vi "MUX - Switch Control.vi"() -> ()   [LabVIEW 2013]
doc: "Sample numeric display item."
uses:
  <vilib>/NI Veristand/Display Template Support/Display Template Support.llb/cluster_Screen Item Settings.ctl
  <vilib>/NI Veristand/Display Template Support/Display Template Support.llb/cluster_Graph Scale Settings.ctl
  <vilib>/NI Veristand/Display Template Support/Display Template Support.llb/cluster_Graph Plot Settings.ctl
  NationalInstruments.VeriStand.SystemStorage
  SubVIs/Relay Data.ctl
  SubVIs/Switch.ctl
  <vilib>/NI Veristand/Display Template Support/Display Template Support.llb/enum_Display Template Handler Minimal To Widget Msg.ctl
  <vilib>/NI Veristand/Display Template Support/Display Template Support.llb/enum_Display Template Handler Minimal To Workspace.ctl
  <vilib>/NI Veristand/Display Template Support/Display Template Support.llb/sub_Display Template Handler Custom.vi
  <vilib>/NI Veristand/Execution/Workspace/NI_VS Workspace ExecutionAPI.lvlib
  MUX Custom Device.lvlib
panel:
  out "MUX Name":string
  in  "Open":bool
  in  "Relays":T1[](array[typedef])
  in  "NIVS.Gateway IP Address":string
  in  "NIVS.System Definition Root":refnum<k24>
  in  "Item.Data":T3
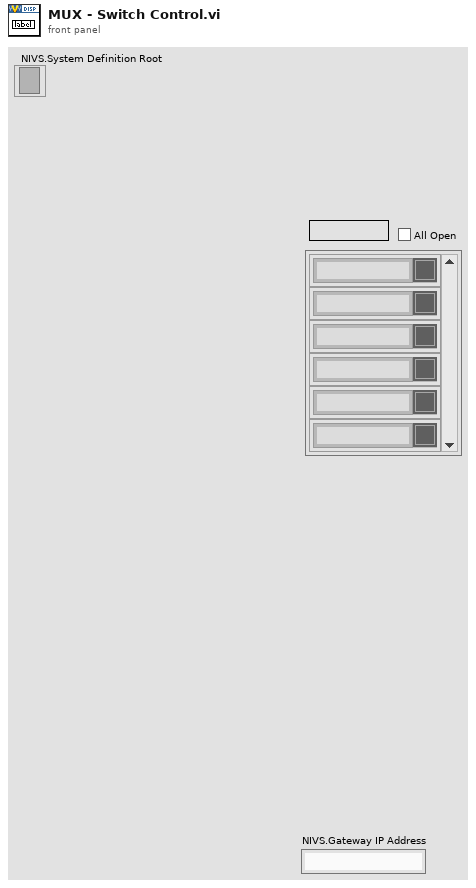
[diagram p1: front panel]
types:
  T1 = typedef "MUX Custom Device.lvlib/Relay Data.ctl" = cluster{"Relay Name":string, "State":T2}
  T2 = typedef "MUX Custom Device.lvlib/Switch.ctl" = bool
  T3 = typedef "cluster_Screen Item Settings.ctl" = cluster{"Template VI":string, "Position X":i32, "Position Y":i32, "Custom":string, "Show Title Bar":bool, "ID":i32, "Always On Top":bool, "Allow Resize":bool, "Allow Minimize":bool, "Allow Close":bool, "Size to Screen":bool, "Screen.ID":i32, "State":enum16{"Normal", "New"}, "Title":string, "Window Bounds":cluster{"[0]":i16, "[1]":i16, "[2]":i16, "[3]":i16}, "Channel Ref":u64, "Unit":string, "Default Units?":bool, "Flash Limit?":bool, "Color 1":u32, "Color 2":u32, "Color 3":u32, "Color 4":u32, "Bck Color":u32, "Fore Color":u32, "Limit 1":dbl, "Limit 2":dbl, "Limit 3":dbl, "Limit 4":dbl, "Limit Mode 1":i32, "Limit Mode 2":i32, "Limit Mode 3":i32, "Limit Mode 4":i32, "Scale Precision":i32, "Scale Min":dbl, "Scale Max":dbl, "Format":i32, "Precision":i32, "Background Type":i32, "IDs":i32[], "Units":string[], "Labels":string[], "Scale Factor":dbl, "Scale Offset":dbl, "YScale Index":u32[], "XScale":T4, "YScales":T4[], "Plots":T5[], "Update Period":dbl, "History Length":dbl, "My.Ref":refnum<vi>, "Is Control?":bool, "Channel Paths":string[], "Custom Data":variant}
  T4 = typedef "cluster_Graph Scale Settings.ctl" = cluster{"Format":u8, "Precision":u8, "Fit":u8, "Label":string, "Use Default Label":bool, "Label Visible":bool, "Min":dbl, "Max":dbl}
  T5 = typedef "cluster_Graph Plot Settings.ctl" = cluster{"Bar Style":u8, "Fill To":i16, "Fill/PtColor":u32, "Line Style":u8, "Line Width":u8, "Color":u32, "Interp":u8, "Point Style":u8}
  T6 = typedef "enum_Display Template Handler Minimal To Workspace.ctl" = cluster{"Operation":enum16{"SetCustomData", "DeleteItem"}, "Data":variant}
  T7 = typedef "enum_Display Template Handler Minimal To Widget Msg.ctl" = enum16{"Stop", "LaunchConfigDialog"}
  T8 = typedef "NI_VS Workspace ExecutionAPI.lvlib/WorkspaceAPI.ctl" = refnum<k24>
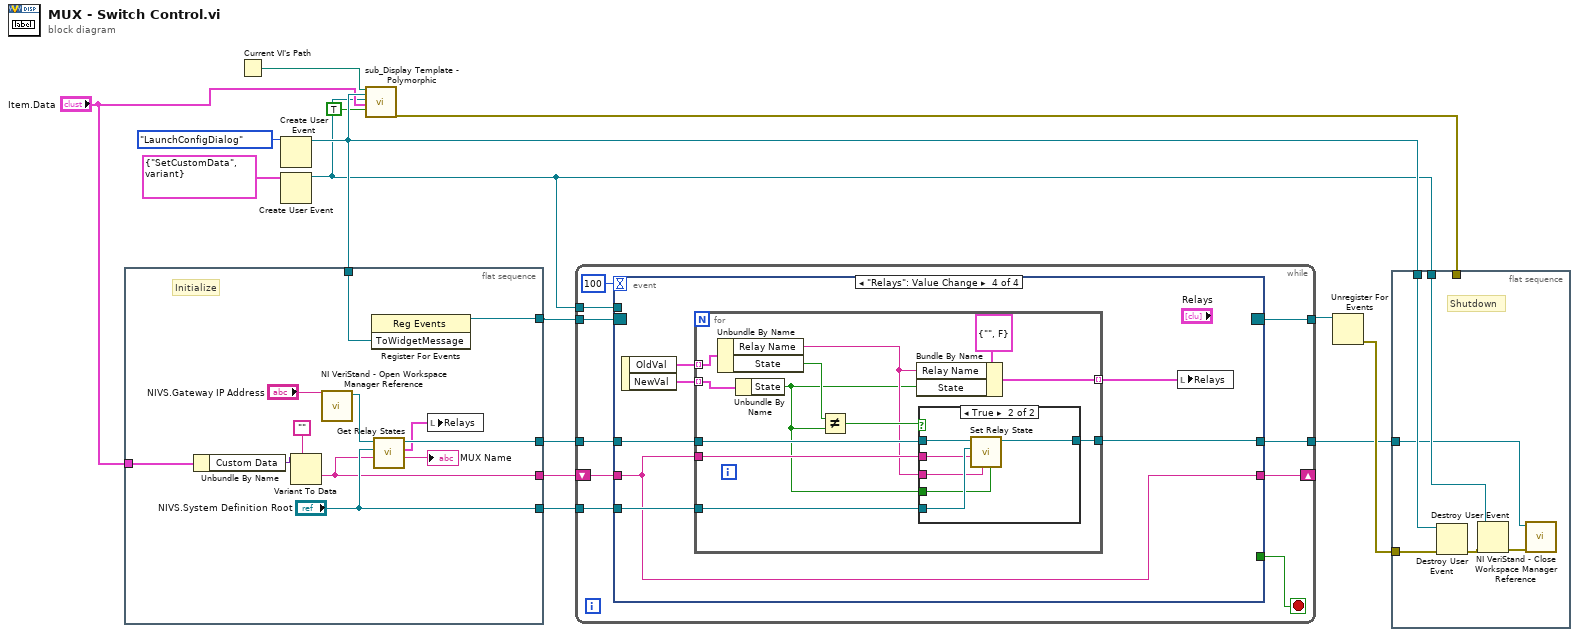
[diagram p0: block diagram]
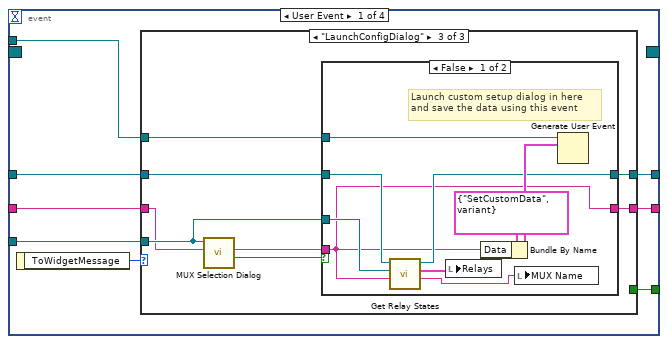
[diagram p2: hidden frame]
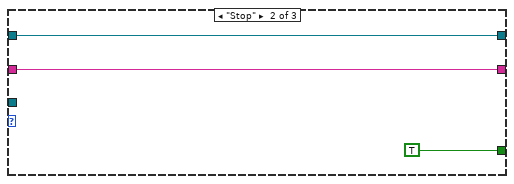
[diagram p4: hidden frame]
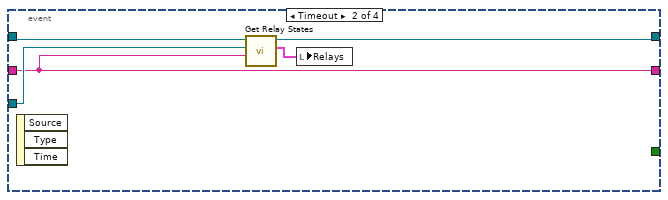
[diagram p6: hidden frame]
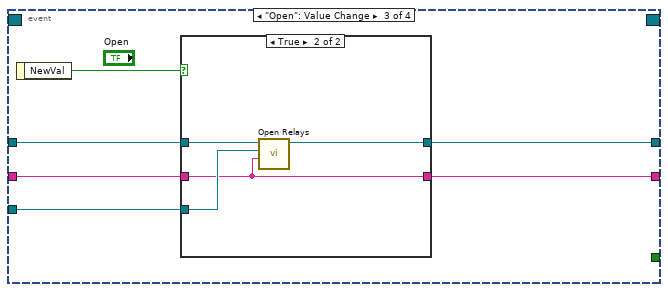
[diagram p7: hidden frame]
diagram:
  n1 = flat-sequence {
    tunnel: [w17] -> w13
    tunnel: w10 -> [w27]
    tunnel: "Item.Data" -> [w26]
    tunnel: ["NIVS.System Definition Root"] -> w4
    tunnel: [w19] -> w3
    tunnel: [w21] -> w2
    frame #0 {
      # "Initialize"
      n2 = Unbundle By Name(w26) -> ("Custom Data"=w25:variant)
      n3 = Variant To Data(type="", Variant=w25) -> (data=w19:string)  [unwired: 1 in, 1 out]
      n4 = call <vilib>:"NI VeriStand - Open Workspace Manager Reference.vi"("Gateway IP Address (\"\": localhost)"="NIVS.Gateway IP Address") -> ("WorkspaceManager"=w22:T8)  [unwired: 9 in, 1 out]
      n5 = register-events(w27) -> (reference out=w17:refnum<event-registration>)  [unwired: 2 in, 1 out]
      n6 = call "Get Relay States.vi"("nodePath"=w19, "NIVS.System Definition Root"="NIVS.System Definition Root", "WorkspaceManager in"=w22) -> ("MUX Name"=→"MUX Name":string, "Relays"=w18:T1[], "WorkspaceManager out"=w21:T8)  [unwired: 5 in, 1 out]
      n7 = local write "Relays"(w18) -> ()
    }
  }
  n8 = Current VI's Path() -> (path=w8:path)
  n9 = Create User Event(user event datatype=enum_Display_Template_Handler_Minimal_To_Widget_Msg."LaunchConfigDialog" ("ToWidgetMessage")) -> (user event=w10:refnum<user-event>)  [unwired: 1 in, 1 out]
  n10 = Create User Event(user event datatype=T6 {"Operation"=enum."SetCustomData", "Data"=variant} ("Data")) -> (user event=w6:refnum<user-event>)  [unwired: 1 in, 1 out]
  n11 = call-poly <vilib>:"sub_Display Template - Polymorphic.vi"("Parent.Path"=w8, "ToWidgetEvent"=w10, "ToWorkspace"=w6, "Item.Data"="Item.Data", "Resizable"=TRUE) -> ("error out"=w15:errorcluster)  [unwired: 1 in, 13 out]
  n12 = while {
    tunnel: w13 -> [w37]
    tunnel: [w35] -> w12
    tunnel: w6 -> [w34]
    tunnel: w4 -> [w33]
    tunnel: w2 -> [w31]
    tunnel: [w30] -> w1
    shift-right: [w28] -> _
    shift-left: w3 -> [w32]
    stop <- w36 stop-if-true
    n13 = event shown="[3] \"Relays\": Value Change" {
      selector: w37 -> [_ _ _ _]
      dyn-events: [_ _ _ _] -> w35
      timeout: 100 -> [_ _ _ _]
      tunnel: [w44 _ _ _] -> w36
      tunnel: w34 -> [w43 _ _ _]
      tunnel: w33 -> [w42 w73 w78 w89]
      tunnel: w32 -> [w41 w70 w77 w88]
      tunnel: w31 -> [w40 w74 w79 w90]
      tunnel: [w39 w72 w76 w87] -> w30
      tunnel: [w38 w70 w75 w88] -> w28
      event User Event {
        n14 = event-data() -> ("ToWidgetMessage"=w45:T7)  [unwired: 1 out]
        n15 = case shown="\"LaunchConfigDialog\"" w45 {
          tunnel: [_ TRUE _] -> w44
          tunnel: w43 -> [_ _ w58]
          tunnel: w42 -> [_ _ w55]
          tunnel: w41 -> [w46 w48 w51]
          tunnel: w40 -> [w47 w49 w54]
          tunnel: [w47 w49 w53] -> w39
          tunnel: [w46 w48 w52] -> w38
          frame Default {
          }
          frame "Stop" {
          }
          frame "LaunchConfigDialog" {
            n16 = call "MUX Selection Dialog.vi"("Current selection"=w51, "NIVS.System Definition Root"=w55) -> ("Cancelled"=w56:bool, "New selection"=w57:string)  [unwired: 7 in, 1 out]
            n17 = case shown="False" w56 {
              tunnel: w58 -> [w67 _]
              tunnel: w57 -> [w60 w68]
              tunnel: w55 -> [w64 _]
              tunnel: w54 -> [w63 w69]
              tunnel: [w61 w69] -> w53
              tunnel: [w60 w68] -> w52
              frame False {
                # "Launch custom setup dialog in here\nand save the data using this event"
                n18 = call "Get Relay States.vi"("nodePath"=w60, "NIVS.System Definition Root"=w64, "WorkspaceManager in"=w63) -> ("MUX Name"=w59:string, "Relays"=w62:T1[], "WorkspaceManager out"=w61:T8)  [unwired: 5 in, 1 out]
                n19 = local write "Relays"(w62) -> ()
                n20 = Bundle By Name(cluster=T6 {"Operation"=enum."SetCustomData", "Data"=variant} ("event data"), "Data"=w60) -> (w65:T6)
                n21 = local write "MUX Name"(w59) -> ()
                n22 = Generate User Event(user event=w67, event data cluster=w65) -> ()  [unwired: 2 in, 2 out]
              }
              frame True {
              }
            }
          }
        }
      }
      event Timeout {
        n23 = event-data() -> ()  [unwired: 4 out]
        n24 = call "Get Relay States.vi"("nodePath"=w70, "NIVS.System Definition Root"=w73, "WorkspaceManager in"=w74) -> ("Relays"=w71:T1[], "WorkspaceManager out"=w72:T8)  [unwired: 5 in, 2 out]
        n25 = local write "Relays"(w71) -> ()
      }
      event "Open": Value Change {
        n26 = event-data() -> ("NewVal"=w80:bool)  [unwired: 1 out]
        n27 = case shown="True" w80 {
          tunnel: w79 -> [w82 w86]
          tunnel: w78 -> [_ w85]
          tunnel: w77 -> [w81 w83]
          tunnel: [w82 w84] -> w76
          tunnel: [w81 w83] -> w75
          frame False {
          }
          frame True {
            n28 = call "Open Relays.vi"("nodePath"=w83, "NIVS.System Definition Root"=w85, "WorkspaceManager in"=w86) -> ("WorkspaceManager out"=w84:T8)  [unwired: 7 in, 1 out]
          }
        }
      }
      event "Relays": Value Change {
        n29 = event-data() -> ("OldVal"=w92:T1[], "NewVal"=w93:T1[])  [unwired: 1 out]
        n30 = for {
          tunnel: w93 -> [w104] mode=indexing
          tunnel: w92 -> [w105] mode=indexing
          tunnel: [w101] -> w91 mode=indexing
          tunnel: w90 -> [w99]
          tunnel: w89 -> [w98]
          tunnel: w88 -> [w97]
          tunnel: [w94] -> w87
          n31 = Unbundle By Name(w105) -> ("Relay Name"=w96:string, "State"=w103:T2)
          n32 = Unbundle By Name(w104) -> ("State"=w95:T2)
          n33 = Not Equal?(x=w103, y=w95) -> (x != y?=w100:T2)
          n34 = Bundle By Name(cluster=T1 {"Relay Name"="", "State"=FALSE} ("Relay Data"), "Relay Name"=w96, "State"=w95) -> (w101:T1)
          n35 = case shown="True" w100 {
            tunnel: w99 -> [w106 w112]
            tunnel: w98 -> [_ w111]
            tunnel: w97 -> [_ w110]
            tunnel: w96 -> [_ w109]
            tunnel: w95 -> [_ w108]
            tunnel: [w106 w107] -> w94
            frame False {
            }
            frame True {
              n36 = call "Set Relay State.vi"("State"=w108, "Relay Name"=w109, "nodePath"=w110, "NIVS.System Definition Root"=w111, "WorkspaceManager in"=w112) -> ("WorkspaceManager out"=w107:T8)  [unwired: 5 in, 1 out]
            }
          }
        }
        n37 = local write "Relays"(w91) -> ()
      }
    }
  }
  n38 = Unregister For Events(event registration refnum=w12) -> (error out=w11:errorcluster)  [unwired: 1 in]
  n39 = flat-sequence {
    tunnel: w15 -> [_]
    tunnel: w11 -> [w117]
    tunnel: w10 -> [w118]
    tunnel: w6 -> [w115]
    tunnel: w1 -> [w113]
    frame #0 {
      # "Shutdown"
      n40 = Destroy User Event(user event=w118, error in=w117) -> (error out=w116:errorcluster)
      n41 = Destroy User Event(user event=w115, error in=w116) -> (error out=w114:errorcluster)
      n42 = call <vilib>:"NI VeriStand - Close Workspace Manager Reference.vi"("error in (no error)"=w114, "WorkspaceManager"=w113) -> ()  [unwired: 9 in, 1 out]
    }
  }
